vi "Create ToastFromXML.vi"(8 "error in (no error)":errorcluster, 10 "XML Stirng":string) -> (0 "error out":errorcluster, 3 "ToastFromXML out":refnum<class "ToastFromXML.lvclass">)   [LabVIEW 2026, in "ToastNotification.lvlib" / "ToastFromXML.lvclass"]
doc: "Create a ToastFromXML source from XML text and retain its WinRT XML Document. Skipped on incoming error. The caller owns Close; class copies share the document reference. Parses XML without guaranteeing toast-schema or Windows-rendering validity. Service initialization and callback registration are separate. Partial-failure cleanup during construction still requires hardening."
uses:
  ToastFromXML.lvclass
  ToastFromXML.lvclass/ToastFromXML.ctl
  Write XML Document.vi
  Toast Native/Toast Native.lvlib
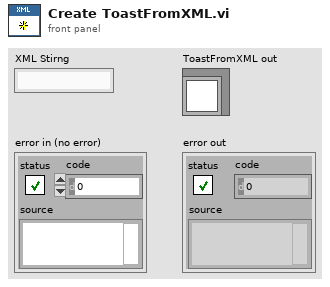
[diagram p1: front panel]
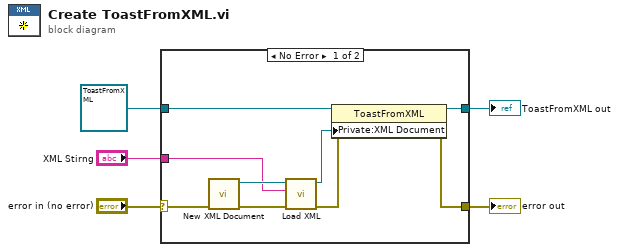
[diagram p0: block diagram]
diagram:
  n1 = case shown="No Error" "error in (no error)" {
    selector: "error in (no error)" -> [w13 w16]
    tunnel: [w7 w16] -> w4
    tunnel: [w9 w15] -> w2
    tunnel: refnum<class "ToastFromXML.lvclass"> refnum ("ToastFromXML") -> [w14 w15]
    tunnel: "XML Stirng" -> [w10 _]
    frame No Error {
      n2 = call "New XML Document.vi"("error in"=w13) -> ("error out"=w12:errorcluster, "XML Document"=w11:refnum<k24>)  [unwired: 9 in]
      n3 = call "Load XML.vi"("error in"=w12, "XML"=w10, "XML Document in"=w11) -> ("error out"=w8:errorcluster, "XML Document out"=w6:refnum<k24>)  [unwired: 7 in]
      n4 = property class="ToastFromXML"(reference=w14, error in=w8, "Private:XML Document"=w6) -> (reference out=w9:refnum<class "ToastFromXML.lvclass">, error out=w7:errorcluster)
    }
    frame Error {
    }
  }
  "error out" <- w4
  "ToastFromXML out" <- w2
